vi "Resolve Value.vi"(4 "Value Name":string, 6 "Namespace":string, 7 "Folder":path, 8 "error in (no error)":errorcluster, 9 "Locals in":refnum<class "Value Tree.lvclass">, 11 "BasicTemplater in":refnum<class "BasicTemplater.lvclass">) -> (0 "error out":errorcluster, 2 "Value":refnum<class "Value Tree.lvclass">, 3 "BasicTemplater out":refnum<class "BasicTemplater.lvclass">)   [LabVIEW 2020, in "HTTP Server.lvlib" / "BasicTemplater.lvclass"]
uses:
  BasicTemplater.lvclass
  C:/dev/lv20CE/relink/lv-http-server/HTTP Server/TemplateService/TemplateService.lvclass
  Value Tree/Value Tree.lvclass
  BasicTemplater.lvclass/BasicTemplater.ctl
  TemplateService/TemplateService.lvclass
  TemplateVariableResolver/TemplateValueResolver.lvclass
  C:/dev/lv20CE/relink/lv-http-server/HTTP Server/Service/Service.lvclass
  C:/dev/lv20CE/relink/lv-http-server/HTTP Server/BasicTemplater/BasicTemplater.lvclass
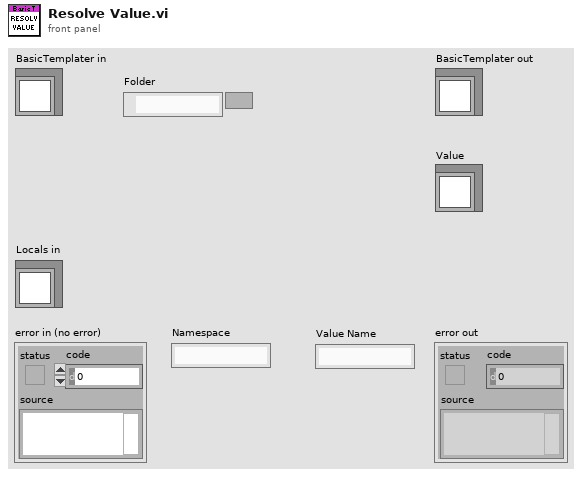
[diagram p1: front panel]
types:
  T1 = map{string, refnum<class "TemplateValueResolver.lvclass">}
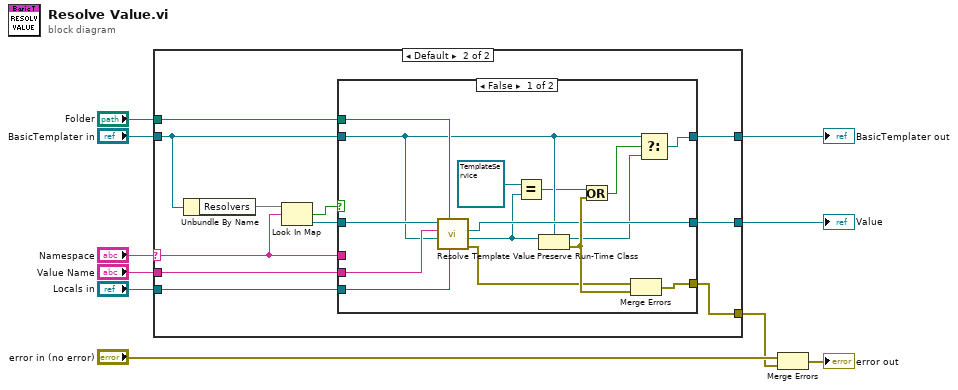
[diagram p0: block diagram]
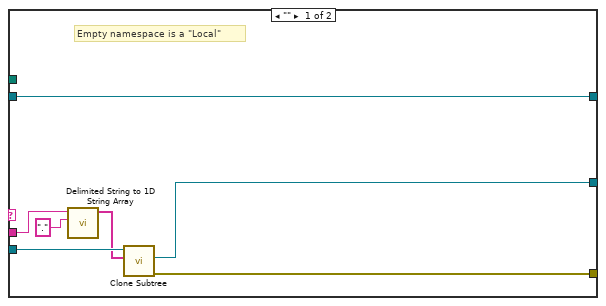
[diagram p2: hidden frame]
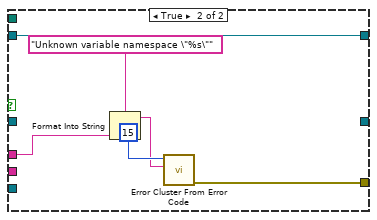
[diagram p3: hidden frame]
diagram:
  n1 = case shown="Default" "Namespace" {
    selector: "Namespace" -> [_ w27]
    tunnel: "Value Name" -> [w13 w26]
    tunnel: [w11 w25] -> w1
    tunnel: [w15 w24] -> w7
    tunnel: "BasicTemplater in" -> [w16 w21]
    tunnel: [w16 w20] -> w5
    tunnel: "Folder" -> [_ w19]
    tunnel: "Locals in" -> [w17 w18]
    frame "" {
      # "Empty namespace is a \"Local\""
      n2 = call <vilib>:"Delimited String to 1D String Array.vi"("delimiter"=".", "delimited string"=w13) -> ("string array"=w12:string[])  [unwired: 9 in]
      n3 = call "Clone Subtree.vi"("Hierarchy"=w12, "Value Tree in"=w17) -> ("error out"=w15:errorcluster, "Subtree"=w11:refnum<class "Value Tree.lvclass">)  [unwired: 7 in, 1 out]
    }
    frame Default {
      n4 = Unbundle By Name(w21) -> ("Resolvers"=w28:T1)
      n5 = Look In Map(map=w28, key=w27) -> (key not found?=w23:bool, value=w22:refnum<class "TemplateValueResolver.lvclass">)  [unwired: 1 in]
      n6 = case shown="False" w23 {
        tunnel: w22 -> [w41 _]
        tunnel: w27 -> [_ w46]
        tunnel: w26 -> [w40 _]
        tunnel: [w39 _] -> w25
        tunnel: [w34 w49] -> w24
        tunnel: w21 -> [w37 w44]
        tunnel: [w35 w44] -> w20
        tunnel: w19 -> [w38 _]
        tunnel: w18 -> [w29 _]
        frame False {
          n7 = call-dynamic "Resolve Template Value.vi"("Locals"=w29, "Folder"=w38, "Template Service in"=w37, "Value Name"=w40, "TemplateVariableResolver in"=w41) -> ("error out"=w42:errorcluster, "Template Service"=w33:refnum<class "TemplateService.lvclass">, "Value"=w39:refnum<class "Value Tree.lvclass">)  [unwired: 4 in]
          n8 = Equal?(x=refnum<class "TemplateService.lvclass"> refnum, y=w33) -> (x = y?=w31:bool)
          n9 = Preserve Run-Time Class(object in=w33, 2:w37) -> (object out=w36:refnum<class "BasicTemplater.lvclass">, error out=w43:errorcluster)  [unwired: 1 in]
          n10 = Or(x=w31, y=w43) -> (x .or. y?=w30:bool)
          n11 = Merge Errors(w42, w43) -> (w34:errorcluster)
          n12 = Select(t=w37, s=w30, f=w36) -> (s? t:f=w35:refnum<class "BasicTemplater.lvclass">)
        }
        frame True {
          n13 = Format Into String(format string="Unknown variable namespace \"%s\"", w46) -> (resulting string=w45:string)  [unwired: 2 in, 1 out]
          n14 = call <vilib>:"Error Cluster From Error Code.vi"("error message (\"\")"=w45, "error code (0)"=15) -> ("error out"=w49:errorcluster)  [unwired: 7 in]
        }
      }
    }
  }
  "BasicTemplater out" <- w5
  "Value" <- w1
  n15 = Merge Errors("error in (no error)", w7) -> (→"error out":errorcluster)
